vi "DiffDriveTrainSim_KitBotWheelSize.vi"(11 "Wheel Size":T1) -> (1 "WheelRadius_M":dbl, 3 "WheelDiameter_M":dbl)   [LabVIEW 2019, in "Trajectory_Library.lvlib"]
doc: "Convience function to allow user to select kit bot wheels size from an enum selector and return the diameter in meters.\n\nInput:\n - Wheel Size -- Enumerated heel size selector\n\nOutput:\n - WheelDiameter_M -- Wheel diameter in meters.\n - WheelRadius_M -- Wheel radius in meters."
uses:
  Trajectory_Library.lvlib
  Enum/DIFF_DRIVE_KitBot_WheelSize_ENUM.ctl
  Conv_Inches_Meters.vi
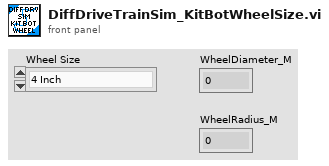
[diagram p1: front panel]
types:
  T1 = typedef "Trajectory_Library.lvlib/DIFF_DRIVE_KitBot_WheelSize_ENUM.ctl" = enum16{"4 Inch", "6 Inch", "8 Inch", "10 Inch"}
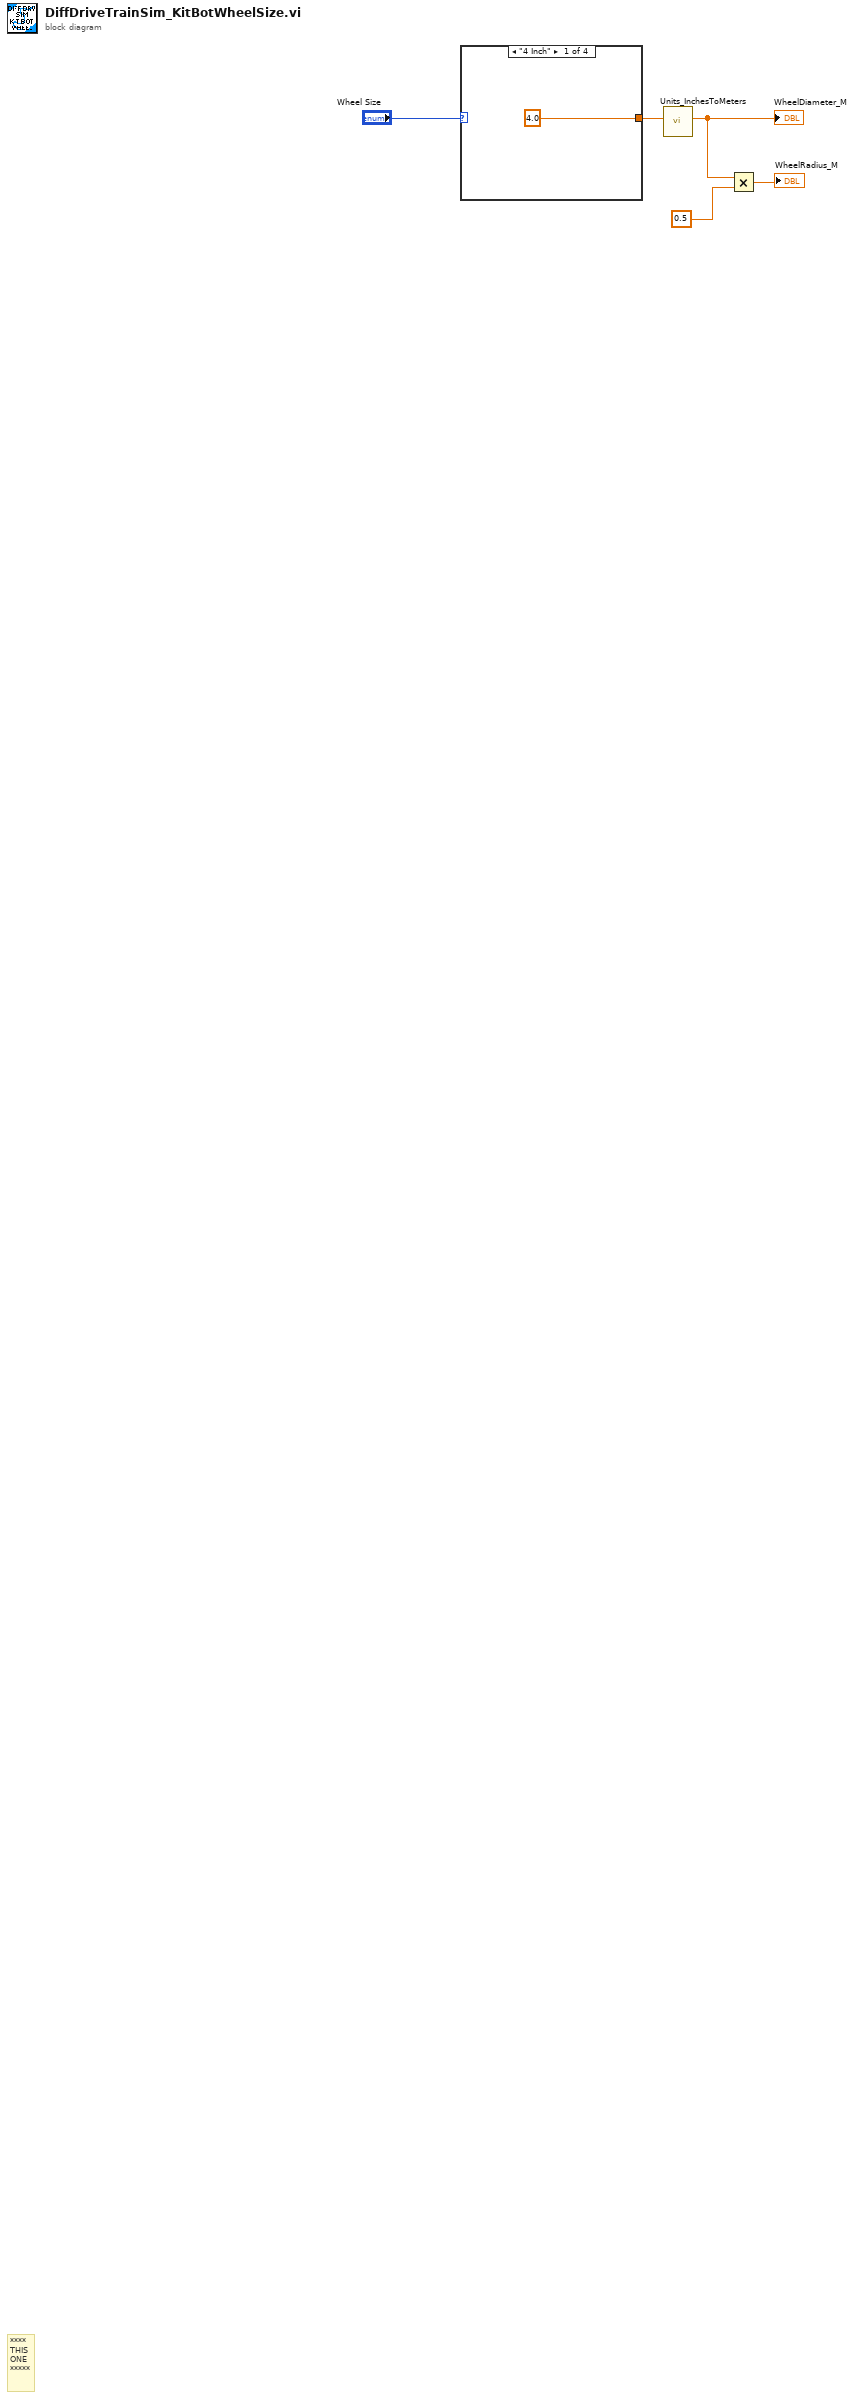
[diagram p0: block diagram]
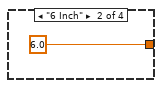
[diagram p2: hidden frame]
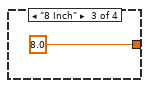
[diagram p3: hidden frame]
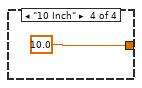
[diagram p4: hidden frame]
diagram:
  # "****\nTHIS\nONE\n*****"
  n1 = case shown="\"4 Inch\"" "Wheel Size" {
    tunnel: [4.0 6.0 8.0 10.0] -> w4
    frame "4 Inch" {
    }
    frame "6 Inch" {
    }
    frame "8 Inch" {
    }
    frame "10 Inch" {
    }
  }
  n2 = call "Units_InchesToMeters.vi"("Inches"=w4) -> ("Meters"=w2:dbl)  [unwired: 10 in]
  "WheelDiameter_M" <- w2
  n3 = Multiply(x=w2, y=0.5) -> (x*y=→"WheelRadius_M":dbl)
